vi "Module Init.vi"(8 "error in (no error)":errorcluster, 11 "DAQmxAI in":refnum<class "DAQmxAI.lvclass">) -> (0 "error out":errorcluster, 3 "DAQmxAI out":refnum<class "DAQmxAI.lvclass">)   [LabVIEW 2020, in "VolatusDAQ.lvlib" / "DAQmxAI.lvclass"]
uses:
  DAQmxAI.lvclass
  C:/dev/lv20CE/relink/lv-volatus/Volatus/Module/Module.lvclass
  DAQmxAI.lvclass/DAQmxAI.ctl
  Volatus/Module/Module.lvclass/Module.ctl
  Volatus/MessageQ/MessageQ.lvclass/MessageQ.ctl
  Volatus/Module/Self Q.vi
  Volatus/MessageQ/Send.vi
  Volatus/Module/Module.lvclass
  VolatusData/Data Processor Module/Data Processor Module.lvclass
  VolatusDAQ.lvlib
  C:/dev/lv20CE/relink/lv-volatus/VolatusDAQ/DAQmxAI/DAQmxAI.lvclass
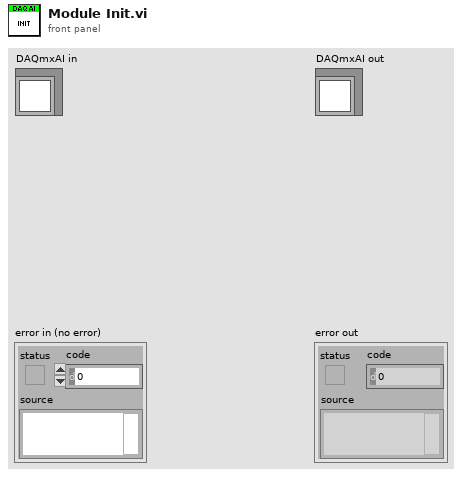
[diagram p1: front panel]
types:
  T1 = typedef "VolatusDAQConfig.lvlib/Sampling Config.ctl" = cluster{"Rate":dbl, "Chunk Size":i32}
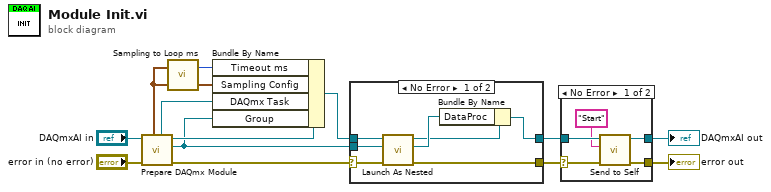
[diagram p0: block diagram]
diagram:
  n1 = call "Prepare DAQmx Module.vi"("error in (no error)"="error in (no error)", "Module in"="DAQmxAI in") -> ("error out"=w5:errorcluster, "Group"=w3:refnum<class "Group.lvclass">, "Module out"=w7:refnum<class "DAQmxAI.lvclass">, "DAQmx Task"=w4:refnum<k21>, "Sampling Config"=w2:T1)  [unwired: 4 in, 1 out]
  n2 = call "Sampling to Loop ms.vi"("Sampling Config"=w2) -> ("Loop Timeout ms"=w1:u32)  [unwired: 6 in]
  n3 = Bundle By Name(cluster=w7, "Timeout ms"=w1, "Sampling Config"=w2, "DAQmx Task"=w4, "Group"=w3) -> (w6:refnum<class "DAQmxAI.lvclass">)
  n4 = case shown="No Error" w5 {
    selector: w5 -> [w19 w21]
    tunnel: w6 -> [w20 w22]
    tunnel: [w15 w21] -> w13
    tunnel: [w16 w22] -> w11
    tunnel: w3 -> [w14 _]
    frame No Error {
      n5 = call "Launch As Nested.vi"("error in (no error)"=w19, "Group"=w14, "Parent in"=w20) -> ("error out"=w15:errorcluster, "MessageQ"=w18:refnum<class "MessageQ.lvclass">, "Parent out"=w17:refnum<class "DAQmxAI.lvclass">)  [unwired: 6 in]
      n6 = Bundle By Name(cluster=w17, "DataProc"=w18) -> (w16:refnum<class "DAQmxAI.lvclass">)
    }
    frame Error {
    }
  }
  n7 = case shown="No Error" w13 {
    selector: w13 -> [w27 w29]
    tunnel: [w26 w29] -> w12
    tunnel: w11 -> [w25 w28]
    tunnel: [w24 w28] -> w10
    frame No Error {
      n8 = call "Send to Self.vi"("error in (no error)"=w27, "Message ID"="Start", "Module in"=w25) -> ("error out"=w26:errorcluster, "Module out"=w24:refnum<class "DAQmxAI.lvclass">)  [unwired: 7 in]
    }
    frame Error {
    }
  }
  "error out" <- w12
  "DAQmxAI out" <- w10
